vi "Save CSV.vi"(5 "CSV FILE PATH Ref":refnum<vi>, 7 "MONITOR TABLE Ref":refnum<vi>, 8 "error in (no error)":errorcluster, 11 "Measurement UI Queue":refnum<queue>) -> (0 "error out":errorcluster)   [LabVIEW 2025, in "I2C Bus Monitor UI.lvlib"]
uses:
  I2C Bus Monitor UI.lvlib
  <vilib>/Utility/file.llb/Write Delimited Spreadsheet (string).vi
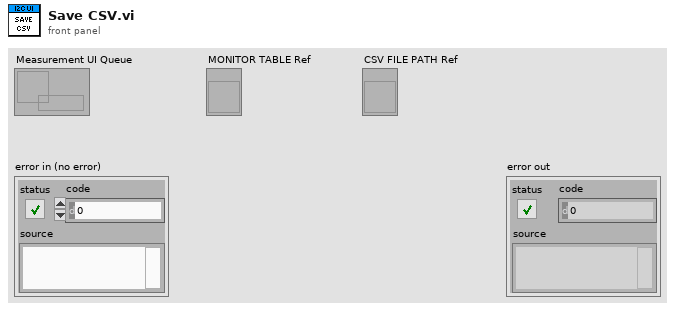
[diagram p1: front panel]
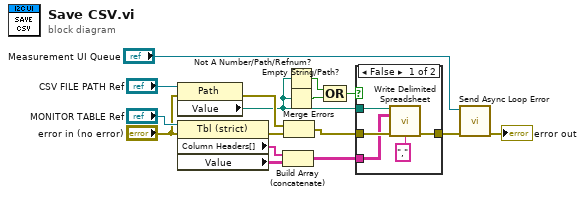
[diagram p0: block diagram]
diagram:
  n1 = property class="Path"(reference="CSV FILE PATH Ref", error in="error in (no error)") -> (error out=w13:errorcluster, "Value"=w4:path)  [unwired: 1 out]
  n2 = property class="Tbl (strict)"(reference="MONITOR TABLE Ref", error in="error in (no error)") -> (error out=w12:errorcluster, "Column Headers[]"=w8:string[], "Value"=w9:string[][])  [unwired: 1 out]
  n3 = Build Array (concatenate)(w8, w9) -> (w10:string[][])
  n4 = Merge Errors(w13, w12) -> (w11:errorcluster)
  n5 = Not A Number/Path/Refnum?(number/path/refnum=w4) -> (NaN/Path/Refnum?=w5:bool)
  n6 = Empty String/Path?(string/path=w4) -> (empty?=w7:bool)
  n7 = Compound Arithmetic op=OR(w5, w7) -> (w6:bool)
  n8 = case shown="False" w6 {
    tunnel: w4 -> [w21 _]
    tunnel: w11 -> [w20 w22]
    tunnel: [w18 w22] -> w3
    tunnel: w10 -> [w17 _]
    frame False {
      n9 = call-poly <vilib>:"Write Delimited Spreadsheet.vi"("file path (dialog if empty)"=w21, "2D data"=w17, "error in (no error)"=w20, "delimiter (\\t)"="," ("delimiter (\\t)")) -> ("error out"=w18:errorcluster)  [unwired: 10 in, 1 out]
    }
    frame True {
    }
  }
  n10 = call "Send Async Loop Error.vi"("error in (no error)"=w3, "Measurement UI Queue"="Measurement UI Queue") -> ("error out"=→"error out":errorcluster)  [unwired: 9 in]
